vi "DoHandshake.vi"(0 "WebSocket Connection in":refnum<k5>, 5 "Supported Protocols (any)":string[](array[string]), 7 "Resource Names":string[](array[string]), 9 "timeout ms (5000)":i32=5000, 11 "error in (no error)":errorcluster, 12 "Additional Return headers (none)":T1[](array[typedef])) -> (4 "WebSocket Connection out":refnum<k5>, 6 "Headers Out":variant, 8 "Resource Name":string, 10 "Request URI":string, 14 "Host":string, 15 "error out":errorcluster)   [LabVIEW 2021, in "LV WebSockets.lvlib"]
doc: "Performs the WebSockets HTTP handshaking on the new TCP connection. The client sends HTTP headers and the server must reply with a correctly formed HTTP response. The VI handles an incoming WS-Protocol and will return it in the response headers if it matches the supported protocols input. Additional HTTP headers can also be returned.\nWebSockets 1.6.0.22\nSam Sharp - MediaMongrels Ltd\nCopyright (c) 2016, MediaMongrels Ltd"
uses:
  LV WebSockets.lvlib
  Headers.ctl
  HTTPResponseCodes.ctl
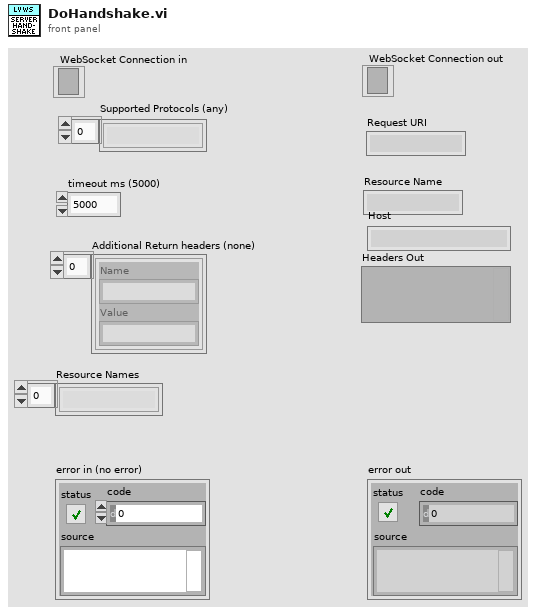
[diagram p1: front panel]
types:
  T1 = typedef "LV WebSockets.lvlib/Headers.ctl" = cluster{"Name":string, "Value":string}
  T2 = typedef "LV WebSockets.lvlib/HTTPResponseCodes.ctl" = u16
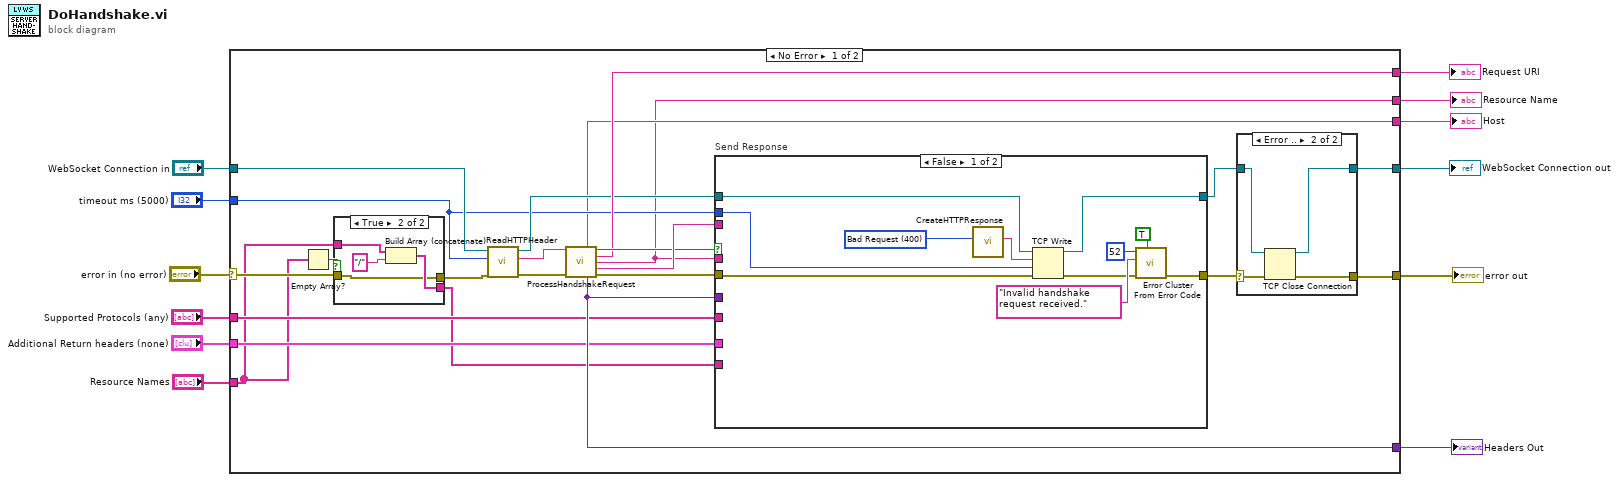
[diagram p0: block diagram]
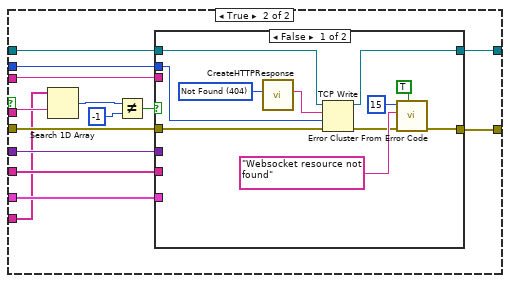
[diagram p4: hidden frame]
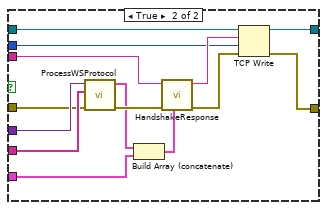
[diagram p5: hidden frame]
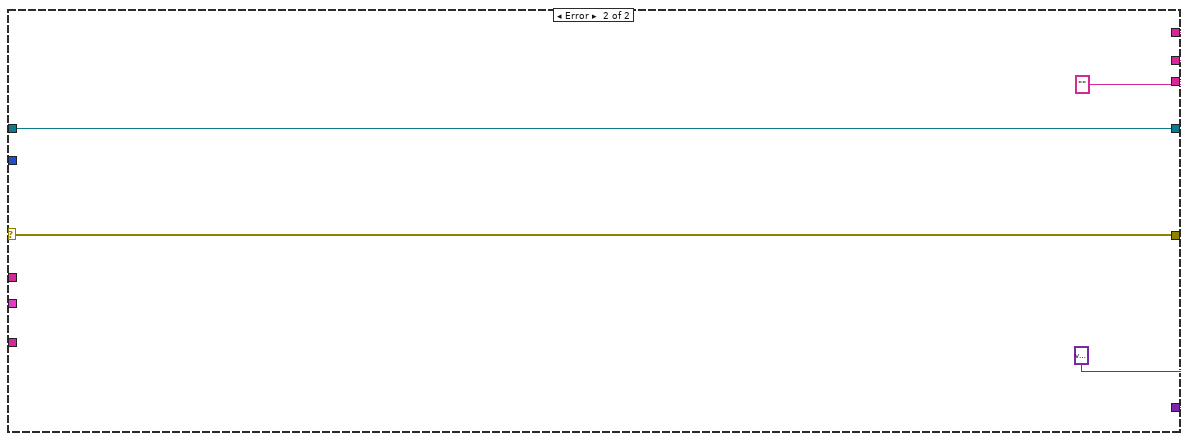
[diagram p6: hidden frame]
diagram:
  n1 = case shown="No Error" "error in (no error)" {
    selector: "error in (no error)" -> [w20 w101]
    tunnel: [w14 w100] -> w12
    tunnel: "WebSocket Connection in" -> [w31 w100]
    tunnel: [w16 w101] -> w9
    tunnel: "timeout ms (5000)" -> [w28 _]
    tunnel: [w26 variant ("Headers Out")] -> w7
    tunnel: [w32 w98] -> w6
    tunnel: "Supported Protocols (any)" -> [w25 _]
    tunnel: "Additional Return headers (none)" -> [w24 _]
    tunnel: [w22 w98] -> w3
    tunnel: [w23 w98] -> w2
    tunnel: "Resource Names" -> [w19 _]
    frame No Error {
      n2 = Empty Array?(array=w19) -> (empty?=w21:bool)
      n3 = case shown="True" w21 {
        tunnel: w20 -> [w42 w44]
        tunnel: [w43 w47] -> w18
        tunnel: w19 -> [w43 w45]
        tunnel: [w42 w44] -> w17
        frame False {
        }
        frame True {
          n4 = Build Array (concatenate)(w45, "/" ("name")) -> (w47:string[])
        }
      }
      n5 = call "ReadHTTPHeader.vi"("error in (no error)"=w17, "timeout ms (25000)"=w28, "WebSocket Connection in"=w31) -> ("error out"=w30:errorcluster, "HTTP Header"=w27:string, "WebSocket Connection out"=w29:refnum<k5>)  [unwired: 6 in]
      n6 = call "ProcessHandshakeRequest.vi"("HTTP Headers"=w27, "error in (no error)"=w30) -> ("Host"=w23:string, "Is Websocket Request?"=w34:bool, "URI"=w32:string, "Resource Name"=w22:string, "Sec-WebSocket-Key"=w35:string, "Headers Out"=w26:variant, "error out"=w33:errorcluster)  [unwired: 7 in]
      n7 = case "Send Response" shown="False" w34 {
        tunnel: w35 -> [_ w72]
        tunnel: w29 -> [w49 w71]
        tunnel: [w48 w70] -> w15
        tunnel: w33 -> [w53 w63]
        tunnel: [w58 w69] -> w13
        tunnel: w28 -> [w50 w68]
        tunnel: w26 -> [_ w67]
        tunnel: w25 -> [_ w66]
        tunnel: w24 -> [_ w65]
        tunnel: w22 -> [_ w64]
        tunnel: w18 -> [_ w59]
        frame False {
          w54 = T2 400 items=["Switching Protocols"=101, "Bad Request"=400, "Forbidden"=403, "Not Found"=404, "Upgrade Required"=426] ("Http Response Codes")
          n8 = call "CreateHTTPResponse.vi"("Http Response Codes"=w54) -> ("Http Response"=w51:string)  [unwired: 10 in]
          n9 = TCP Write(connection ID=w49, data in=w51, error in (no error)=w53, 9:w50) -> (connection ID out=w48:refnum<k5>, error out=w52:errorcluster)  [unwired: 1 out]
          n10 = call <vilib>:"Error Cluster From Error Code.vi"("show call chain? (False)"=TRUE, "error in (no error)"=w52, "error message (\"\")"="Invalid handshake request received." ("error message (\"\")"), "error code (0)"=52) -> ("error out"=w58:errorcluster)  [unwired: 5 in]
        }
        frame True {
          n11 = Search 1D Array(1D array=w59, element=w64) -> (index of element=w61:i32)  [unwired: 1 in]
          n12 = Not Equal?(x=w61, y=-1) -> (x != y?=w62:bool)
          n13 = case shown="False" w62 {
            tunnel: w72 -> [_ w97]
            tunnel: w71 -> [w80 w95]
            tunnel: [w79 w94] -> w70
            tunnel: [w74 w92] -> w69
            tunnel: w68 -> [w78 w91]
            tunnel: w67 -> [_ w89]
            tunnel: w66 -> [_ w87]
            tunnel: w65 -> [_ w85]
            tunnel: w63 -> [w81 w84]
            frame False {
              w83 = T2 404 items=["Switching Protocols"=101, "Bad Request"=400, "Forbidden"=403, "Not Found"=404, "Upgrade Required"=426] ("Http Response Codes")
              n14 = call "CreateHTTPResponse.vi"("Http Response Codes"=w83) -> ("Http Response"=w82:string)  [unwired: 10 in]
              n15 = TCP Write(connection ID=w80, data in=w82, error in (no error)=w81, 9:w78) -> (connection ID out=w79:refnum<k5>, error out=w73:errorcluster)  [unwired: 1 out]
              n16 = call <vilib>:"Error Cluster From Error Code.vi"("show call chain? (False)"=TRUE, "error in (no error)"=w73, "error message (\"\")"="Websocket resource not found" ("error message (\"\")"), "error code (0)"=15) -> ("error out"=w74:errorcluster)  [unwired: 5 in]
            }
            frame True {
              n17 = call "ProcessWSProtocol.vi"("error in (no error)"=w84, "Supported Protocols (any)"=w87, "Headers In"=w89) -> ("error out"=w90:errorcluster, "Protocol Header"=w88:T1[])  [unwired: 7 in]
              n18 = Build Array (concatenate)(w88, w85) -> (w86:T1[])
              n19 = call "HandshakeResponse.vi"("additional headers (none)"=w86, "error in (no error)"=w90, "Sec-WebSocket-Key"=w97) -> ("error out"=w93:errorcluster, "Response Headers"=w96:string)  [unwired: 7 in]
              n20 = TCP Write(connection ID=w95, data in=w96, error in (no error)=w93, 9:w91) -> (connection ID out=w94:refnum<k5>, error out=w92:errorcluster)  [unwired: 1 out]
            }
          }
        }
      }
      n21 = case shown="Error .." w13 {
        selector: w13 -> [w36 w41]
        tunnel: w15 -> [w37 w40]
        tunnel: [w37 w39] -> w14
        tunnel: [w36 w38] -> w16
        frame No Error {
        }
        frame Error {
          n22 = TCP Close Connection(connection ID=w40, error in (no error)=w41) -> (connection ID out=w39:refnum<k5>, error out=w38:errorcluster)  [unwired: 1 in]
        }
      }
    }
    frame Error {
      w98 = "" ("Path")
    }
  }
  "WebSocket Connection out" <- w12
  "error out" <- w9
  "Headers Out" <- w7
  "Request URI" <- w6
  "Resource Name" <- w3
  "Host" <- w2
